vi "Initialize UI.vi"(8 "error in (no error)":errorcluster, 10 "Control Refs":T2, 11 "node ref in":T1) -> (0 "error out":errorcluster, 2 "Linux?":bool, 3 "node ref out":T1)   [LabVIEW 2015, in "TDMS datalogger editor node.lvclass"]
uses:
  TDMS datalogger editor node.lvclass
  <vilib>/NI/Configuration Framework/Node/NodeRef.ctl
  <vilib>/NI/Configuration Framework/Node/NISE_CEF_Node.lvclass
  Control Refs.ctl
  module/configuration/TDMS datalogger configuration.lvclass
  TDMS datalogger editor node.lvclass/TDMS datalogger editor node.ctl
  module/configuration/TDMS datalogger configuration.lvclass/TDMS datalogger configuration.ctl
  module/configuration/Write log directory.vi
  module/configuration/Write backup directory.vi
  Write channel table.vi
  Write avail tags table.vi
  module/configuration/Read backup directory.vi
  module/configuration/Read log directory.vi
  module/configuration/Read queue size.vi
  module/configuration/Read scans per write.vi
  module/configuration/Read add enable channel.vi
  module/configuration/Read channel pattern matches.vi
  module/configuration/Read log name.vi
  module/configuration/Read logrotate_options.vi
  module/configuration/Read log file path.vi
  <vilib>/NI/DCAF/Tag Editor Core/Configuration Editor/Classes/Module editor node/Read Module Configuration.vi
  <vilib>/NI/DCAF/Tag Editor Core/Configuration Editor/Classes/Module editor node/Write Module Configuration.vi
  <vilib>/NI/Tag Bus Module Framework/module configuration/TBM module configuration.lvclass
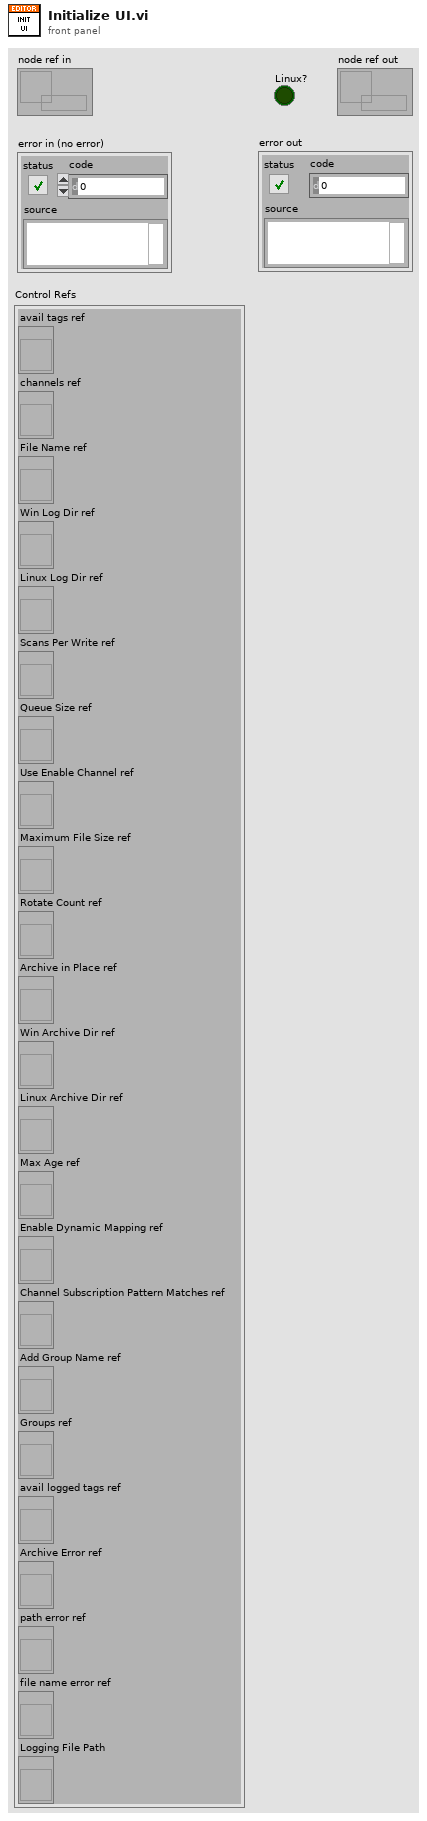
[diagram p1: front panel]
types:
  T1 = typedef "NISE_CEF_Node.lvclass/NodeRef.ctl" = refnum<data-value>
  T2 = typedef "Control Refs.ctl" = cluster{"avail tags ref":refnum<vi>, "channels ref":refnum<vi>, "File Name ref":refnum<vi>, "Win Log Dir ref":refnum<vi>, "Linux Log Dir ref":refnum<vi>, "Scans Per Write ref":refnum<vi>, "Queue Size ref":refnum<vi>, "Use Enable Channel ref":refnum<vi>, "Maximum File Size ref":refnum<vi>, "Rotate Count ref":refnum<vi>, "Archive in Place ref":refnum<vi>, "Win Archive Dir ref":refnum<vi>, "Linux Archive Dir ref":refnum<vi>, "Max Age ref":refnum<vi>, "Enable Dynamic Mapping ref":refnum<vi>, "Channel Subscription Pattern Matches ref":refnum<vi>, "Add Group Name ref":refnum<vi>, "Groups ref":refnum<vi>, "avail logged tags ref":refnum<vi>, "Archive Error ref":refnum<vi>, "path error ref":refnum<vi>, "file name error ref":refnum<vi>, "Logging File Path":refnum<vi>}
  T3 = typedef "TBM configuration.lvclass/Target Types.ctl" = enum16{"Windows", "Mac", "Linux", "Linux RT ARM", "VxWorks", "Pharlap", "Other", "Linux RT x64"}
  T4 = typedef "LogRotate.lvclass/options.ctl" = cluster{"max file size (bytes)":i64, "rotate count":u32, "max age (days)":dbl, "No archive dir":bool, "Archive dir":path}
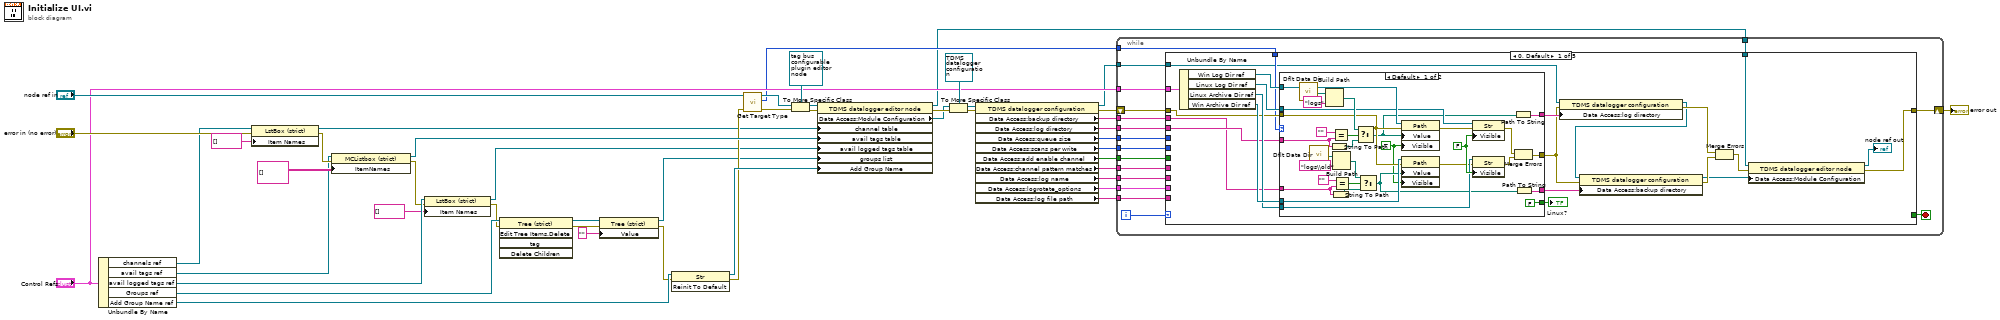
[diagram p0: block diagram]
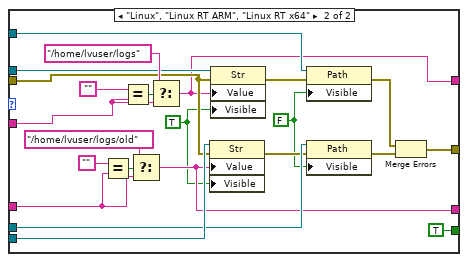
[diagram p2: hidden frame]
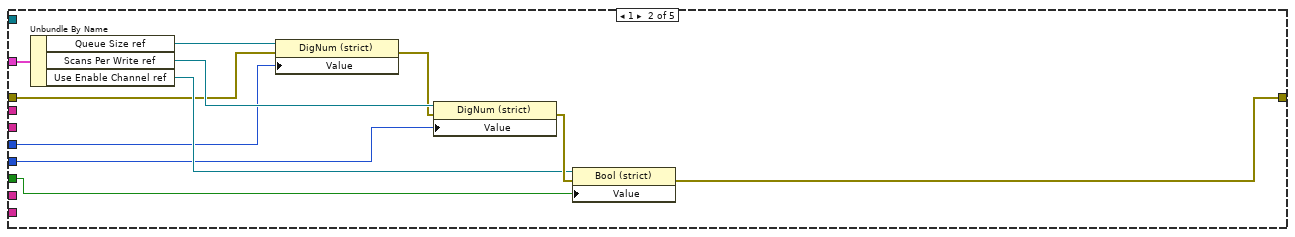
[diagram p3: hidden frame]
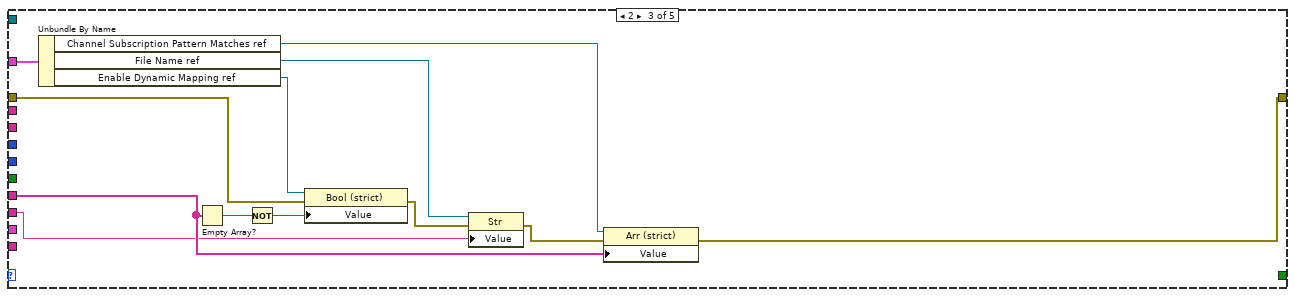
[diagram p4: hidden frame]
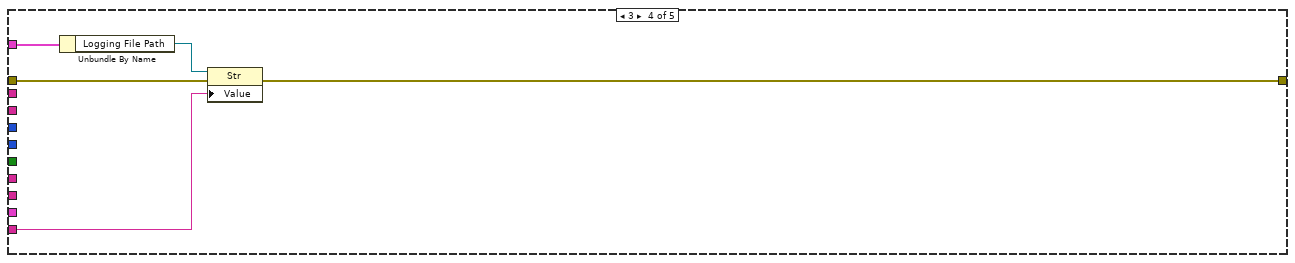
[diagram p5: hidden frame]
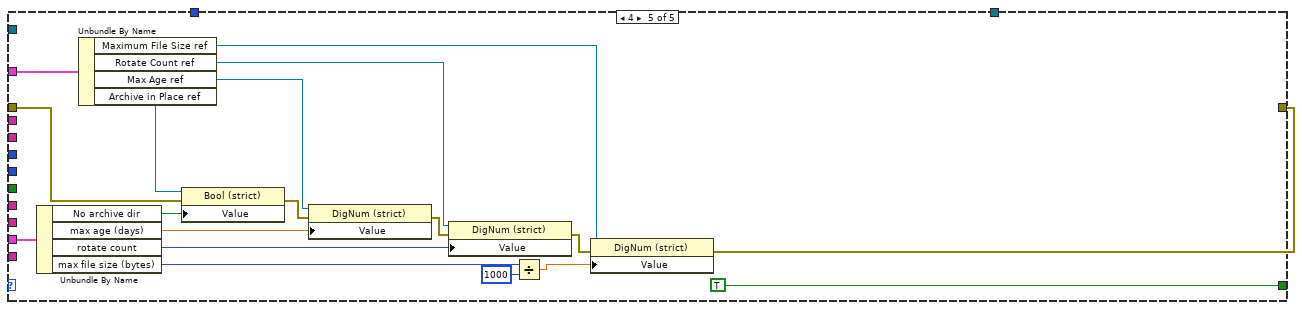
[diagram p6: hidden frame]
diagram:
  n1 = Unbundle By Name("Control Refs") -> ("channels ref"=w29:refnum<vi>, "avail tags ref"=w28:refnum<vi>, "avail logged tags ref"=w8:refnum<vi>, "Groups ref"=w27:refnum<vi>, "Add Group Name ref"=w26:refnum<vi>)
  n2 = property on="Property Node" class="LstBox (strict)"(reference=w29, error in="error in (no error)", "Item Names"=string[] []) -> (reference out=w25:refnum<vi>, error out=w32:errorcluster)
  n3 = property on="Property Node" class="MCListbox (strict)"(reference=w28, error in=w32, "ItemNames"=string[][] [] ("Item Names")) -> (reference out=w34:refnum<vi>, error out=w7:errorcluster)
  n4 = property on="Property Node" class="LstBox (strict)"(reference=w8, error in=w7, "Item Names"=string[] []) -> (reference out=w5:refnum<vi>, error out=w6:errorcluster)
  n5 = invoke class="Tree (strict)" method="Edit Tree Items.Delete"(reference=w27, error in=w6) -> (reference out=w23:refnum<vi>, error out=w24:errorcluster)  [unwired: 3 in, 3 out]
  n6 = property on="Property Node" class="Tree (strict)"(reference=w23, error in=w24, "Value"="" ("Groups")) -> (reference out=w22:refnum<vi>, error out=w21:errorcluster)
  n7 = invoke class="Str" method="Reinit To Default"(reference=w26, error in=w21) -> (reference out=w33:refnum<vi>, error out=w31:errorcluster)  [unwired: 1 in, 1 out]
  n8 = call "Get Target Type.vi"("error in (no error)"=w31, "node ref in"="node ref in") -> ("error out"=w38:errorcluster, "Target Type"=w16:T3, "node ref out"=w37:T1)  [unwired: 6 in]
  n9 = To More Specific Class(target class=refnum<data-value> refnum ("data value reference"), reference=w37, error in=w38) -> (specific class reference=w41:refnum<data-value>, error out=w40:errorcluster)
  n10 = property class="TDMS datalogger editor node"(reference=w41, error in=w40, "channel table"=w25, "avail tags table"=w34, "avail logged tags table"=w5, "groups list"=w22, "Add Group Name"=w33) -> (reference out=w3:refnum<data-value>, error out=w48:errorcluster, "Data Access:Module Configuration"=w46:refnum<class "TBM module configuration.lvclass">)
  n11 = To More Specific Class(target class=refnum<class "TDMS datalogger configuration.lvclass"> refnum ("TDMS datalogger configuration"), reference=w46, error in=w48) -> (specific class reference=w44:refnum<class "TDMS datalogger configuration.lvclass">, error out=w47:errorcluster)
  n12 = property class="TDMS datalogger configuration"(reference=w44, error in=w47) -> (reference out=w2:refnum<class "TDMS datalogger configuration.lvclass">, error out=w17:errorcluster, "Data Access:backup directory"=w18:string, "Data Access:log directory"=w19:string, "Data Access:queue size"=w15:u16, "Data Access:scans per write"=w13:u16, "Data Access:add enable channel"=w14:bool, "Data Access:channel pattern matches"=w12:string[], "Data Access:log name"=w11:string, "Data Access:logrotate_options"=w10:T4, "Data Access:log file path"=w1:string)
  n13 = while {
    tunnel: "Control Refs" -> [w63]
    tunnel: w19 -> [w62]
    tunnel: w18 -> [w61]
    shift-right: [w60] -> w9
    shift-left: w17 -> [w59]
    tunnel: w16 -> [w58]
    tunnel: w15 -> [w57]
    tunnel: w13 -> [w56]
    tunnel: w14 -> [w55]
    tunnel: w12 -> [w54]
    tunnel: w11 -> [w53]
    tunnel: w10 -> [w52]
    tunnel: w3 -> [w51]
    tunnel: w2 -> [w50]
    tunnel: w1 -> [w49]
    i -> [w64]
    stop <- w65 stop-if-true
    n14 = case shown="0, Default" w64 {
      tunnel: [_ _ _ _ TRUE] -> w65
      tunnel: w63 -> [w87 w152 w162 w169 w185]
      tunnel: w62 -> [w81 _ _ _ _]
      tunnel: w61 -> [w80 _ _ _ _]
      tunnel: [w66 w142 w153 w166 w173] -> w60
      tunnel: w59 -> [w79 w143 w156 w167 w174]
      tunnel: w58 -> [w78 _ _ _ _]
      tunnel: w57 -> [_ w146 _ _ _]
      tunnel: w56 -> [_ w145 _ _ _]
      tunnel: w55 -> [_ w144 _ _ _]
      tunnel: w54 -> [_ _ w158 _ _]
      tunnel: w53 -> [_ _ w157 _ _]
      tunnel: w52 -> [_ _ _ _ w187]
      tunnel: w51 -> [w76 _ _ _ _]
      tunnel: w50 -> [w73 _ _ _ _]
      tunnel: w49 -> [_ _ _ w165 _]
      frame 0, Default {
        n15 = Unbundle By Name(w87) -> ("Win Log Dir ref"=w85:refnum<vi>, "Linux Log Dir ref"=w84:refnum<vi>, "Linux Archive Dir ref"=w82:refnum<vi>, "Win Archive Dir ref"=w83:refnum<vi>)
        n16 = case shown="Default" w78 {
          tunnel: w80 -> [w103 w133]
          tunnel: w81 -> [w111 w138]
          tunnel: [FALSE TRUE] -> w86
          tunnel: w84 -> [w101 w132]
          tunnel: w82 -> [w99 w131]
          tunnel: w85 -> [w102 w130]
          tunnel: w83 -> [w100 w129]
          tunnel: [w96 w125] -> w72
          tunnel: w79 -> [w93 w123]
          tunnel: [w91 w122] -> w74
          tunnel: [w89 w121] -> w75
          frame Default {
            w118 = FALSE ("Visible")
            w88 = TRUE ("Visible")
            n17 = call <vilib>:"Dflt Data Dir.vi"() -> ("App:Default Data Directory"=w114:path)
            n18 = call <vilib>:"Dflt Data Dir.vi"() -> ("App:Default Data Directory"=w106:path)
            n19 = Build Path(base path=w114, name or relative path="logs") -> (appended path=w116:path)
            n20 = String To Path(string=w111) -> (path=w110:path)
            n21 = String To Path(string=w103) -> (path=w109:path)
            n22 = Equal?(x="", y=w111) -> (x = y?=w112:bool)
            n23 = Build Path(base path=w106, name or relative path="logs\\old") -> (appended path=w104:path)
            n24 = Equal?(x="", y=w103) -> (x = y?=w108:bool)
            n25 = Select(t=w116, s=w112, f=w110) -> (s? t:f=w90:path)
            n26 = Select(t=w104, s=w108, f=w109) -> (s? t:f=w92:path)
            n27 = property on="Property Node" class="Path"(reference=w102, error in=w93, "Value"=w90, "Visible"=w88) -> (error out=w94:errorcluster)  [unwired: 1 out]
            n28 = property on="Property Node" class="Path"(reference=w100, error in=w93, "Value"=w92, "Visible"=w88) -> (error out=w98:errorcluster)  [unwired: 1 out]
            n29 = property on="Property Node" class="Str"(reference=w101, error in=w94, "Visible"=w118) -> (error out=w95:errorcluster)  [unwired: 1 out]
            n30 = property on="Property Node" class="Str"(reference=w99, error in=w98, "Visible"=w118) -> (error out=w97:errorcluster)  [unwired: 1 out]
            n31 = Path To String(path=w90) -> (string=w89:string)
            n32 = Merge Errors(w95, w97) -> (w96:errorcluster)
            n33 = Path To String(path=w92) -> (string=w91:string)
          }
          frame "Linux", "Linux RT ARM", "Linux RT x64" {
            w119 = FALSE ("Visible")
            w120 = TRUE ("Visible")
            n34 = Equal?(x="", y=w133) -> (x = y?=w135:bool)
            n35 = Equal?(x="", y=w138) -> (x = y?=w139:bool)
            n36 = Select(t="/home/lvuser/logs/old", s=w135, f=w133) -> (s? t:f=w122:string)
            n37 = Select(t="/home/lvuser/logs", s=w139, f=w138) -> (s? t:f=w121:string)
            n38 = property on="Property Node" class="Str"(reference=w131, error in=w123, "Value"=w122, "Visible"=w120) -> (error out=w128:errorcluster)  [unwired: 1 out]
            n39 = property on="Property Node" class="Str"(reference=w132, error in=w123, "Value"=w121, "Visible"=w120) -> (error out=w127:errorcluster)  [unwired: 1 out]
            n40 = property on="Property Node" class="Path"(reference=w130, error in=w127, "Visible"=w119) -> (error out=w124:errorcluster)  [unwired: 1 out]
            n41 = property on="Property Node" class="Path"(reference=w129, error in=w128, "Visible"=w119) -> (error out=w126:errorcluster)  [unwired: 1 out]
            n42 = Merge Errors(w124, w126) -> (w125:errorcluster)
          }
        }
        "Linux?" <- w86
        n43 = property class="TDMS datalogger configuration"(reference=w73, error in=w72, "Data Access:log directory"=w75) -> (reference out=w69:refnum<class "TDMS datalogger configuration.lvclass">, error out=w71:errorcluster)
        n44 = property class="TDMS datalogger configuration"(reference=w69, error in=w72, "Data Access:backup directory"=w74) -> (reference out=w68:refnum<class "TDMS datalogger configuration.lvclass">, error out=w70:errorcluster)
        n45 = Merge Errors(w71, w70) -> (w67:errorcluster)
        n46 = property class="TDMS datalogger editor node"(reference=w76, error in=w67, "Data Access:Module Configuration"=w68) -> (reference out=→"node ref out":refnum<data-value>, error out=w66:errorcluster)
      }
      frame 1 {
        n47 = Unbundle By Name(w152) -> ("Queue Size ref"=w151:refnum<vi>, "Scans Per Write ref"=w150:refnum<vi>, "Use Enable Channel ref"=w147:refnum<vi>)
        n48 = property on="Property Node" class="DigNum (strict)"(reference=w151, error in=w143, "Value"=w146) -> (error out=w149:errorcluster)  [unwired: 1 out]
        n49 = property class="DigNum (strict)"(reference=w150, error in=w149, "Value"=w145) -> (error out=w148:errorcluster)  [unwired: 1 out]
        n50 = property on="Property Node" class="Bool (strict)"(reference=w147, error in=w148, "Value"=w144) -> (error out=w142:errorcluster)  [unwired: 1 out]
      }
      frame 2 {
        n51 = Unbundle By Name(w162) -> ("Channel Subscription Pattern Matches ref"=w161:refnum<vi>, "File Name ref"=w160:refnum<vi>, "Enable Dynamic Mapping ref"=w159:refnum<vi>)
        n52 = Empty Array?(array=w158) -> (empty?=w163:bool)
        n53 = Not(x=w163) -> (.not. x?=w164:bool)
        n54 = property on="Property Node" class="Bool (strict)"(reference=w159, error in=w156, "Value"=w164) -> (error out=w155:errorcluster)  [unwired: 1 out]
        n55 = property on="Property Node" class="Str"(reference=w160, error in=w155, "Value"=w157) -> (error out=w154:errorcluster)  [unwired: 1 out]
        n56 = property class="Arr (strict)"(reference=w161, error in=w154, "Value"=w158) -> (error out=w153:errorcluster)  [unwired: 1 out]
      }
      frame 3 {
        n57 = Unbundle By Name(w169) -> ("Logging File Path"=w168:refnum<vi>)
        n58 = property on="Property Node" class="Str"(reference=w168, error in=w167, "Value"=w165) -> (error out=w166:errorcluster)  [unwired: 1 out]
      }
      frame 4 {
        n59 = Unbundle By Name(w187) -> ("No archive dir"=w177:bool, "max age (days)"=w176:dbl, "rotate count"=w175:u32, "max file size (bytes)"=w171:i64)
        n60 = Unbundle By Name(w185) -> ("Maximum File Size ref"=w184:refnum<vi>, "Rotate Count ref"=w183:refnum<vi>, "Max Age ref"=w181:refnum<vi>, "Archive in Place ref"=w179:refnum<vi>)
        n61 = property on="Property Node" class="Bool (strict)"(reference=w179, error in=w174, "Value"=w177) -> (error out=w178:errorcluster)  [unwired: 1 out]
        n62 = property on="Property Node" class="DigNum (strict)"(reference=w181, error in=w178, "Value"=w176) -> (error out=w180:errorcluster)  [unwired: 1 out]
        n63 = property on="Property Node" class="DigNum (strict)"(reference=w183, error in=w180, "Value"=w175) -> (error out=w182:errorcluster)  [unwired: 1 out]
        n64 = Divide(x=w171, y=i64 1000) -> (x/y=w170:dbl)
        n65 = property on="Property Node" class="DigNum (strict)"(reference=w184, error in=w182, "Value"=w170) -> (error out=w173:errorcluster)  [unwired: 1 out]
      }
    }
  }
  "error out" <- w9
